vi "SerialSend.vi"(6 "清缓存":bool=TRUE, 8 "error in (no error)":errorcluster caption="错误输入（无错误）", 10 "SendData":string, 11 "PORT":refnum<visa-resource-name>) -> (0 "error out":errorcluster caption="错误输出", 2 "返回数":u32, 3 "PORT out":refnum<visa-resource-name>)   [LabVIEW 2025]
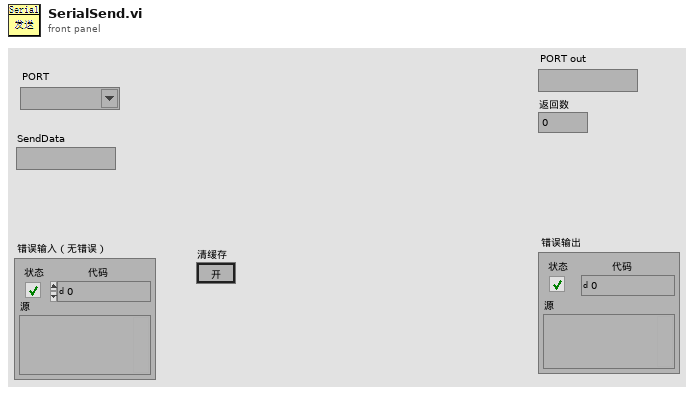
[diagram p1: front panel]
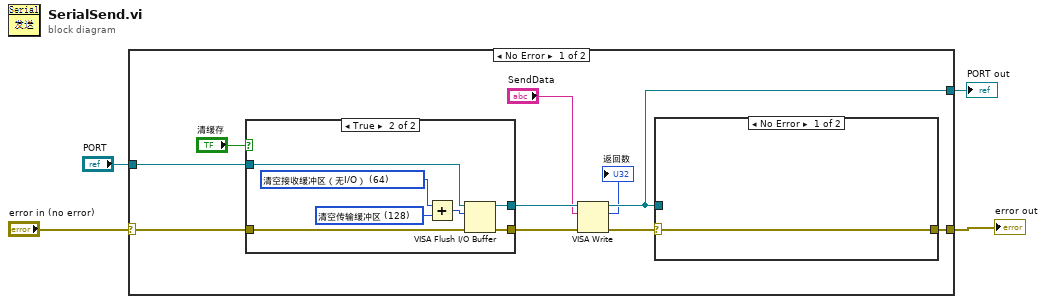
[diagram p0: block diagram]
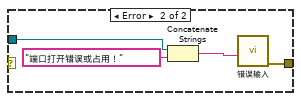
[diagram p3: hidden frame]
diagram:
  n1 = case shown="No Error" "error in (no error)" {
    selector: "error in (no error)" -> [w6 w30]
    tunnel: "PORT" -> [w7 w29]
    tunnel: [w11 w30] -> w3
    tunnel: [w8 w29] -> w1
    frame No Error {
      n2 = case shown="True" "清缓存" {
        tunnel: w7 -> [w16 w17]
        tunnel: [w15 w23] -> w13
        tunnel: [w16 w18] -> w12
        tunnel: w6 -> [w15 w22]
        frame False {
        }
        frame True {
          w21 = u16 128 items=["清空接收缓冲区"=16, "向设备写入传输缓冲区"=32, "清空接收缓冲区（无I/O）"=64, "清空传输缓冲区"=128] ("Mask")
          w20 = u16 64 items=["清空接收缓冲区"=16, "向设备写入传输缓冲区"=32, "清空接收缓冲区（无I/O）"=64, "清空传输缓冲区"=128] ("Mask")
          n3 = Add(x=w20, y=w21) -> (x+y=w19:u16)
          n4 = VISA Flush I/O Buffer(VISA resource name=w17, mask (16)=w19, error in (no error)=w22) -> (VISA resource name out=w18:refnum<visa-resource-name>, error out=w23:errorcluster)
        }
      }
      n5 = VISA Write(VISA resource name=w12, write buffer="SendData", error in (no error)=w13) -> (VISA resource name out=w8:refnum<visa-resource-name>, return count=→"返回数":u32, error out=w14:errorcluster)
      n6 = case shown="No Error" w14 {
        selector: w14 -> [w24 _]
        tunnel: w8 -> [_ w27]
        tunnel: [w24 w25] -> w11
        frame No Error {
        }
        frame Error {
          n7 = Concatenate Strings(w27, "端口打开错误或占用！" ("字符串")) -> (w26:string)
          n8 = call "错误输入.vi"("source"=w26) -> ("error out"=w25:errorcluster)  [unwired: 10 in]
        }
      }
    }
    frame Error {
    }
  }
  "error out" <- w3
  "PORT out" <- w1
